vi "JocAcabatSenseSubvis.vi"() -> ()   [LabVIEW 2023]
uses:
  <vilib>/MakerHub/LINX/Public/Peripherals/Analog/Analog Read N Chans.vi
  <vilib>/MakerHub/LINX/Private/Local IO/LinxAnalogRead.vi
  <vilib>/MakerHub/LINX/Public/Utilities/Check Channel.vi
  <vilib>/MakerHub/LINX/Public/Utilities/Open Serial.vi
  <vilib>/MakerHub/LINX/Private/Utilties/Generate Error.vi
  <vilib>/MakerHub/LINX/LMH-LINX.lvlib
panel:
  out "?":string
  out "?":string="Benvingut a la jungla! El teu objectiu és sobreviure! Per aconseguir-ho, has de caçar les preses (punts verds) i fugir dels depredadors (punts vermells). Alerta, a mida que vagis avançant en el joc, aniràn apreixent més preses i depredadors. Per sort, si t'estàs a punt de quedar sense vides, apareixerà un quadrat groc, si l'atrapes, et proporcionarà una vida extra. També has de tenir en compte que tens 40 s per atrapar les preses, si tardes més, et moriràs de gana... Abans que passi però, apareixerà un diamant groc. Atrapa'l i tindràs una mica més de temps per caçar. Bona sort! "
  out "Nivell:":i32
  in  "base path":path
  in  "Serial Port":refnum<visa-resource-name>="N/A"
  out "Tablero":cluster{dbl[], dbl[]}[](graph)
  out "Vides":i32
  out "Preses capturades":i32
  out "Temps sense menjar (s)":u32
  in  "?":bool
  out "ms totals":u32
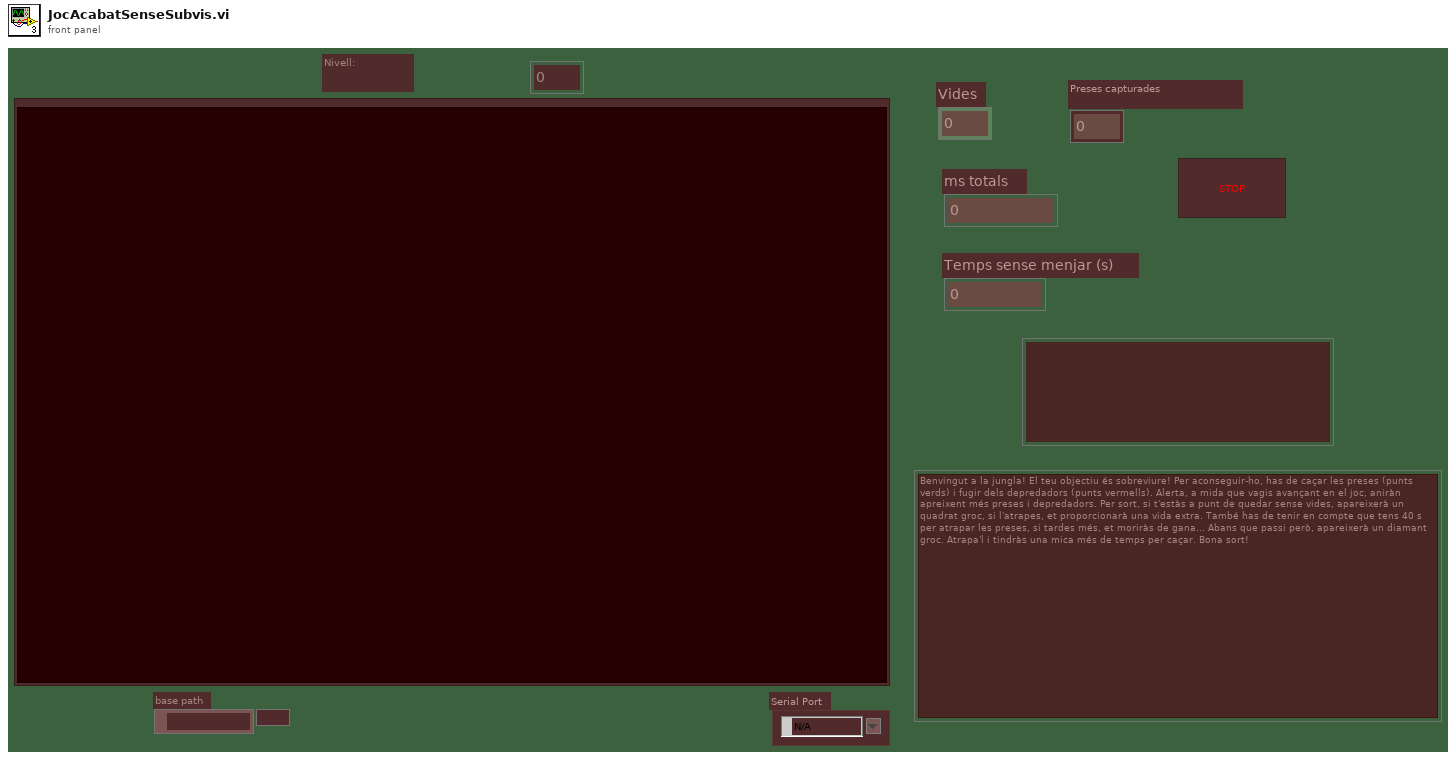
[diagram p1: front panel]
types:
  T1 = enum16{"open", "replace", "create", "open or create", "replace or create", "replace or create with confirmation"}
  T2 = typedef "LMH-LINX.lvlib/LINX Ref.ctl" = cluster{"IO":T3, "Interface":T4, "LINX Device Config":T5}
  T3 = typedef "LMH-LINX.lvlib/Platform.ctl" = enum16{"Remote", "Local"}
  T4 = typedef "LMH-LINX.lvlib/Interface.ctl" = enum16{"Serial", "TCP"}
  T5 = typedef "LMH-LINX.lvlib/Device.lvlib/LINX Device Config.ctl" = cluster{"Interface":T4, "COM Port":refnum<visa-resource-name>, "TCP Configuration":T6, "Device Family":u8, "Device ID":u8, "Device Name":string, "TCP Ref":refnum<k5>, "Channels":T7}
  T6 = typedef "LMH-LINX.lvlib/Device.lvlib/TCP Config.ctl" = cluster{"IP Address":string, "Port":u16}
  T7 = typedef "LMH-LINX.lvlib/Channels.ctl" = cluster{"DI":u8[], "DO":u8[], "AI":u8[], "AO":u8[], "PWM":u8[], "QE":u8[], "UART":u8[], "I2C 2":u8[], "SPI":u8[], "CAN":u8[], "Servo":u8[], "AI Ref (V)":dbl, "AI Resolution (Bits)":u8, "AO Ref (V)":dbl, "AO Resolution (Bits)":u8}
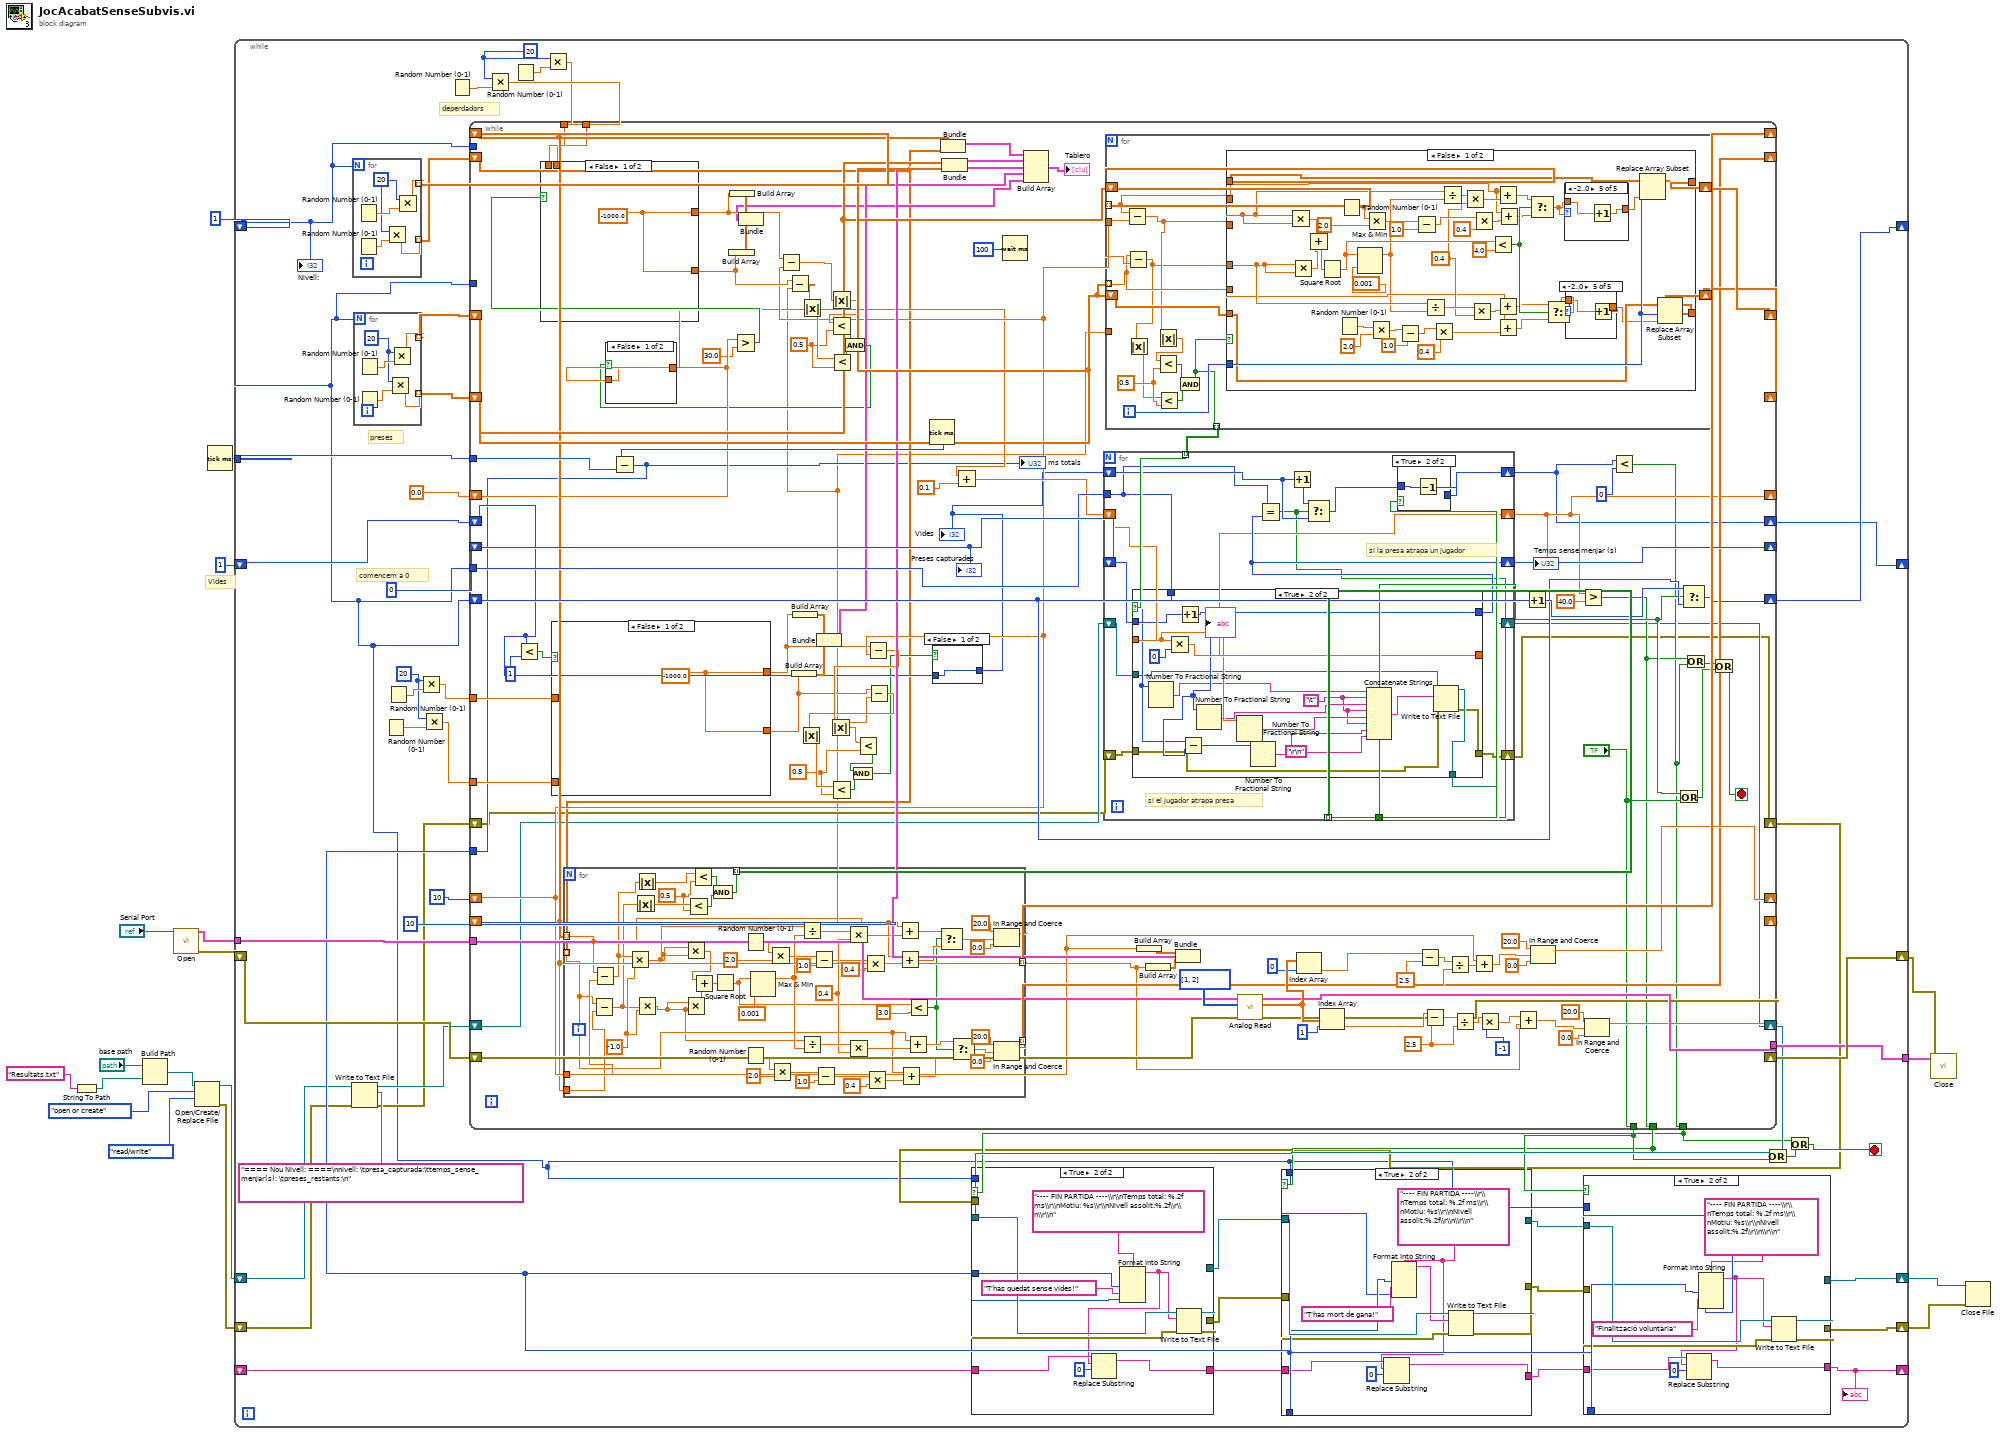
[diagram p0: block diagram]
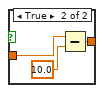
[diagram p5: hidden frame]
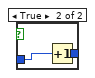
[diagram p6: hidden frame]
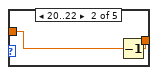
[diagram p8: hidden frame]
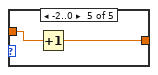
[diagram p11: hidden frame]
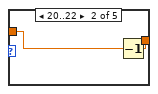
[diagram p12: hidden frame]
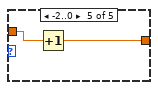
[diagram p15: hidden frame]
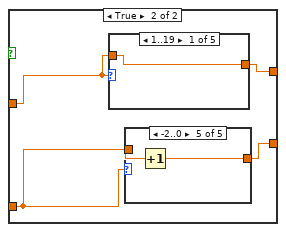
[diagram p16: hidden frame]
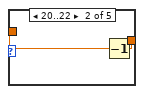
[diagram p18: hidden frame]
diagram:
  # "Vides"
  n1 = String To Path(string="Resultats.txt") -> (path=w3:path)
  n2 = Build Path(base path="base path", name or relative path=w3) -> (appended path=w6:path)
  n3 = call-poly <vilib>:"Open.vi"("Serial Port"="Serial Port") -> ("Error Out"=w12:errorcluster, "LINX Resource"=w13:T2)  [unwired: 8 in, 1 out]
  n4 = Open/Create/Replace File(file path (use dialog)=w6, operation (0:open)=T1."open or create", access (0:read/write)=enum16{"read/write", "read-only", "write-only"}."read/write") -> (refnum out=w9:refnum<file>, error out=w7:errorcluster)  [unwired: 3 in, 1 out]
  n5 = Tick Count (ms)() -> (millisecond timer value=w17:u32)
  n6 = while {
    shift-right: [w63] -> _
    shift-left: 1 -> [w23]
    tunnel: w17 -> [w54]
    shift-right: [w60] -> _
    shift-left: 1 -> [w61]
    tunnel: [w58] -> w14
    tunnel: w13 -> [w57]
    shift-right: [w59] -> w15
    shift-left: w12 -> [w55]
    shift-right: [w25] -> w2
    shift-left: w7 -> [w30]
    shift-right: [w24] -> w1
    shift-left: w9 -> [w33]
    shift-right: [w19] -> _
    shift-left: _ -> [w22]
    stop <- w40 stop-if-true
    w44 = 20
    w47 = 20
    # "comencem a 0"
    # "deperdadors"
    # "preses"
    n7 = Write to Text File(file (use dialog)=w33, text="==== Nou Nivell: ====\nnivell: \tpresa_capturada:\ttemps_sense_menjar(s): \tpreses_restants:\n", error in=w30) -> (refnum out=w34:refnum<file>, error out=w29:errorcluster)  [unwired: 1 in, 1 out]
    n8 = for {
      N: w23 -> [_]
      tunnel: [w450] -> w68 mode=indexing
      tunnel: [w449] -> w67 mode=indexing
      w451 = 20
      n9 = Random Number (0-1)() -> (number: 0 to 1=w453:dbl)
      n10 = Random Number (0-1)() -> (number: 0 to 1=w452:dbl)
      n11 = Multiply(x=w451, y=w452) -> (x*y=w449:dbl)
      n12 = Multiply(x=w451, y=w453) -> (x*y=w450:dbl)
    }
    n13 = for {
      N: w23 -> [_]
      tunnel: [w445] -> w66 mode=indexing
      tunnel: [w444] -> w65 mode=indexing
      w446 = 20
      n14 = Random Number (0-1)() -> (number: 0 to 1=w448:dbl)
      n15 = Random Number (0-1)() -> (number: 0 to 1=w447:dbl)
      n16 = Multiply(x=w446, y=w447) -> (x*y=w444:dbl)
      n17 = Multiply(x=w446, y=w448) -> (x*y=w445:dbl)
    }
    n18 = Random Number (0-1)() -> (number: 0 to 1=w46:dbl)
    n19 = Random Number (0-1)() -> (number: 0 to 1=w45:dbl)
    n20 = Multiply(x=w44, y=w45) -> (x*y=w42:dbl)
    n21 = Multiply(x=w44, y=w46) -> (x*y=w43:dbl)
    n22 = Random Number (0-1)() -> (number: 0 to 1=w51:dbl)
    n23 = Multiply(x=w47, y=w51) -> (x*y=w49:dbl)
    n24 = Random Number (0-1)() -> (number: 0 to 1=w50:dbl)
    n25 = Multiply(x=w47, y=w50) -> (x*y=w48:dbl)
    n26 = while {
      tunnel: w23 -> [_]
      shift-right: [w202] -> _
      shift-left: w68 -> [w163]
      shift-right: [w183] -> _
      shift-left: w67 -> [w125]
      shift-right: [w192] -> _
      shift-left: w66 -> [w186]
      shift-right: [w185] -> _
      shift-left: w65 -> [w193]
      shift-right: [w198] -> _
      shift-left: 10 -> [w140]
      shift-right: [w194] -> _
      shift-left: 10 -> [w114]
      shift-right: [w203] -> w59
      shift-left: w55 -> [w205]
      tunnel: [w204] -> w58
      tunnel: w23 -> [_]
      shift-right: [w170] -> w60
      shift-left: w61 -> [w138]
      shift-right: [w188] -> _
      shift-left: 0 -> [w190]
      tunnel: w23 -> [w184]
      tunnel: [w171] -> w37
      shift-right: [w180] -> w63
      shift-left: w23 -> [w181]
      tunnel: w57 -> [w179]
      tunnel: ["?"] -> w38
      tunnel: w54 -> [w176]
      shift-right: [w173] -> _
      shift-left: 0.0 -> [w135]
      tunnel: [w165] -> w36
      tunnel: w49 -> [w124]
      tunnel: w48 -> [w123]
      tunnel: w43 -> [w122]
      tunnel: w42 -> [w121]
      shift-right: [w118] -> w39
      shift-left: w34 -> [w119]
      tunnel: [w117] -> w35
      shift-right: [w115] -> w28
      shift-left: w29 -> [w116]
      stop <- w166 stop-if-true
      w133 = 0.5
      w132 = 0.5
      w213 = 2.5
      w214 = 2.5
      n27 = Less?(x=w138, y=1) -> (x < y?=w161:bool)
      n28 = case shown="False" w161 {
        tunnel: [w249 w253] -> w129
        tunnel: [w249 w252] -> w139
        tunnel: w122 -> [_ w251]
        tunnel: w121 -> [_ w250]
        frame False {
          w249 = -1000.0
        }
        frame True {
          n29 = case shown="1..19" w250 {
            tunnel: [w261 w263 w264 w265 w267] -> w253
            tunnel: w250 -> [w261 w262 w264 w265 w266]
            frame 1..19 {
            }
            frame 20..22 {
              n30 = Decrement(x=w262) -> (x-1=w263:dbl)
            }
            frame 23.. {
            }
            frame ..-3 {
            }
            frame -2..0 {
              n31 = Increment(x=w266) -> (x+1=w267:dbl)
            }
          }
          n32 = case shown="-2..0" w251 {
            tunnel: [w254 w256 w257 w258 w260] -> w252
            tunnel: w251 -> [w254 w255 w257 w258 w259]
            frame 1..19 {
            }
            frame 20..22 {
              n33 = Decrement(x=w255) -> (x-1=w256:dbl)
            }
            frame 23.. {
            }
            frame ..-3 {
            }
            frame -2..0 {
              n34 = Increment(x=w259) -> (x+1=w260:dbl)
            }
          }
        }
      }
      n35 = for {
        tunnel: w140 -> [w325]
        tunnel: w114 -> [w324]
        tunnel: w125 -> [w319] mode=indexing
        tunnel: w163 -> [w320] mode=indexing
        tunnel: [w323] -> w202 mode=indexing
        tunnel: [w322] -> w183 mode=indexing
        tunnel: [w309] -> w189 mode=indexing
        w312 = 0.5
        w321 = -1.0
        w355 = 0.4
        n36 = Subtract(x=w319, y=w324) -> (x-y=w315:dbl)
        n37 = Subtract(x=w320, y=w325) -> (x-y=w316:dbl)
        n38 = Multiply(x=w316, y=w321) -> (x*y=w318:dbl)
        n39 = Absolute Value(x=w315) -> (abs(x)=w313:dbl)
        n40 = Absolute Value(x=w316) -> (abs(x)=w314:dbl)
        n41 = Multiply(x=w315, y=w321) -> (x*y=w317:dbl)
        n42 = Multiply(x=w318, y=w318) -> (x*y=w362:dbl)
        n43 = Multiply(x=w317, y=w317) -> (x*y=w361:dbl)
        n44 = Less?(x=w313, y=w312) -> (x < y?=w310:bool)
        n45 = Less?(x=w314, y=w312) -> (x < y?=w311:bool)
        n46 = Add(x=w362, y=w361) -> (x+y=w360:dbl)
        n47 = And(x=w311, y=w310) -> (x .and. y?=w309:bool)
        n48 = Square Root(x=w360) -> (sqrt(x)=w326:dbl)
        n49 = Random Number (0-1)() -> (number: 0 to 1=w344:dbl)
        n50 = Random Number (0-1)() -> (number: 0 to 1=w351:dbl)
        n51 = Max & Min(x=w326, y=0.001) -> (max(x,y)=w357:dbl)  [unwired: 1 out]
        n52 = Multiply(x=w344, y=2.0) -> (x*y=w342:dbl)
        n53 = Multiply(x=w351, y=2.0) -> (x*y=w349:dbl)
        n54 = Divide(x=w318, y=w357) -> (x/y=w354:dbl)
        n55 = Divide(x=w317, y=w357) -> (x/y=w356:dbl)
        n56 = Subtract(x=w342, y=1.0) -> (x-y=w340:dbl)
        n57 = Subtract(x=w349, y=1.0) -> (x-y=w347:dbl)
        n58 = Multiply(x=w354, y=w355) -> (x*y=w353:dbl)
        n59 = Multiply(x=w356, y=w355) -> (x*y=w352:dbl)
        n60 = Multiply(x=w340, y=0.4) -> (x*y=w338:dbl)
        n61 = Multiply(x=w347, y=0.4) -> (x*y=w345:dbl)
        n62 = Add(x=w320, y=w353) -> (x+y=w334:dbl)
        n63 = Add(x=w320, y=w338) -> (x+y=w335:dbl)
        n64 = Add(x=w319, y=w345) -> (x+y=w337:dbl)
        n65 = Add(x=w319, y=w352) -> (x+y=w336:dbl)
        n66 = Less?(x=w326, y=3.0) -> (x < y?=w333:bool)
        n67 = Select(t=w334, s=w333, f=w335) -> (s? t:f=w331:dbl)
        n68 = Select(t=w336, s=w333, f=w337) -> (s? t:f=w332:dbl)
        n69 = In Range and Coerce(upper limit=20.0, x=w331, lower limit=0.0) -> (coerced(x)=w323:dbl)  [unwired: 1 out]
        n70 = In Range and Coerce(upper limit=20.0, x=w332, lower limit=0.0) -> (coerced(x)=w322:dbl)  [unwired: 1 out]
      }
      n71 = Greater?(x=w135, y=30.0) -> (0:w157:bool)
      n72 = case shown="False" w157 {
        tunnel: [w230 w234] -> w149
        tunnel: [w230 w233] -> w148
        tunnel: w124 -> [_ w232]
        tunnel: w123 -> [_ w231]
        frame False {
          w230 = -1000.0
        }
        frame True {
          n73 = case shown="1..19" w231 {
            tunnel: [w242 w244 w245 w246 w248] -> w234
            tunnel: w231 -> [w242 w243 w245 w246 w247]
            frame 1..19 {
            }
            frame 20..22 {
              n74 = Decrement(x=w243) -> (x-1=w244:dbl)
            }
            frame 23.. {
            }
            frame ..-3 {
            }
            frame -2..0 {
              n75 = Increment(x=w247) -> (x+1=w248:dbl)
            }
          }
          n76 = case shown="1..19" w232 {
            tunnel: [w235 w237 w238 w239 w241] -> w233
            tunnel: w232 -> [w235 w236 w238 w239 w240]
            frame 1..19 {
            }
            frame 20..22 {
              n77 = Decrement(x=w236) -> (x-1=w237:dbl)
            }
            frame 23.. {
            }
            frame ..-3 {
            }
            frame -2..0 {
              n78 = Increment(x=w240) -> (x+1=w241:dbl)
            }
          }
        }
      }
      n79 = Build Array(w148) -> (w155:dbl[])
      n80 = Build Array(w149) -> (w156:dbl[])
      n81 = Bundle(w156, w155) -> (w131:cluster{dbl[], dbl[]})  [unwired: 1 in]
      n82 = Subtract(x=w149, y=w140) -> (x-y=w147:dbl)
      n83 = Subtract(x=w148, y=w114) -> (x-y=w150:dbl)
      n84 = Build Array(w139) -> (w159:dbl[])
      n85 = Build Array(w129) -> (w160:dbl[])
      n86 = Absolute Value(x=w150) -> (abs(x)=w152:dbl)
      n87 = Bundle(w160, w159) -> (w158:cluster{dbl[], dbl[]})  [unwired: 1 in]
      n88 = Absolute Value(x=w147) -> (abs(x)=w151:dbl)
      n89 = Less?(x=w151, y=w132) -> (x < y?=w154:bool)
      n90 = Less?(x=w152, y=w132) -> (x < y?=w153:bool)
      n91 = And(x=w154, y=w153) -> (x .and. y?=w128:bool)
      n92 = case shown="False" w128 {
        tunnel: w135 -> [w223 w226]
        tunnel: [w223 w224] -> w134
        frame False {
        }
        frame True {
          n93 = Subtract(x=w226, y=10.0) -> (x-y=w224:dbl)
        }
      }
      n94 = Subtract(x=w129, y=w140) -> (x-y=w144:dbl)
      n95 = Absolute Value(x=w144) -> (abs(x)=w143:dbl)
      n96 = Less?(x=w143, y=w133) -> (x < y?=w146:bool)
      n97 = Subtract(x=w139, y=w114) -> (x-y=w142:dbl)
      n98 = Absolute Value(x=w142) -> (abs(x)=w141:dbl)
      n99 = Less?(x=w141, y=w133) -> (x < y?=w145:bool)
      n100 = And(x=w146, y=w145) -> (x .and. y?=w137:bool)
      n101 = Tick Count (ms)() -> (millisecond timer value=w177:u32)
      n102 = Subtract(x=w177, y=w176) -> (x-y=w117:u32)
      "ms totals" <- w117
      n103 = case shown="False" w137 {
        tunnel: w138 -> [w227 w229]
        tunnel: [w227 w228] -> w136
        frame False {
        }
        frame True {
          n104 = Increment(x=w229) -> (x+1=w228:i32)
        }
      }
      "Vides" <- w136
      n105 = Bundle(w163, w125) -> (w191:cluster{dbl[], dbl[]})  [unwired: 1 in]
      n106 = Bundle(w186, w193) -> (w126:cluster{dbl[], dbl[]})  [unwired: 1 in]
      n107 = Add(x=w134, y=0.1) -> (x+y=w174:dbl)
      n108 = Wait (ms)(milliseconds to wait=u32 100) -> ()  [unwired: 1 out]
      n109 = for {
        tunnel: w140 -> [w379]
        tunnel: w114 -> [w374]
        tunnel: w186 -> [w373] mode=indexing
        tunnel: w193 -> [w369] mode=indexing
        shift-right: [w368] -> w192
        shift-left: w186 -> [w372]
        shift-right: [w370] -> w185
        shift-left: w193 -> [w371]
        tunnel: [w363] -> w120 mode=indexing
        i -> [w378]
        w377 = 0.5
        n110 = Subtract(x=w373, y=w379) -> (x-y=w366:dbl)
        n111 = Subtract(x=w369, y=w374) -> (x-y=w364:dbl)
        n112 = Absolute Value(x=w364) -> (abs(x)=w367:dbl)
        n113 = Absolute Value(x=w366) -> (abs(x)=w365:dbl)
        n114 = Less?(x=w365, y=w377) -> (x < y?=w376:bool)
        n115 = Less?(x=w367, y=w377) -> (x < y?=w375:bool)
        n116 = And(x=w376, y=w375) -> (x .and. y?=w363:bool)
        n117 = case shown="False" w363 {
          tunnel: w378 -> [w386 w438]
          tunnel: w373 -> [w391 _]
          tunnel: w369 -> [w393 _]
          tunnel: w366 -> [w392 _]
          tunnel: w364 -> [w394 _]
          tunnel: w372 -> [w390 w442]
          tunnel: w371 -> [w382 w443]
          tunnel: [w389 w441] -> w368
          tunnel: [w388 w440] -> w370
          frame False {
            w397 = 0.4
            n118 = Multiply(x=w392, y=w392) -> (x*y=w404:dbl)
            n119 = Multiply(x=w394, y=w394) -> (x*y=w405:dbl)
            n120 = Add(x=w404, y=w405) -> (x+y=w406:dbl)
            n121 = Square Root(x=w406) -> (sqrt(x)=w407:dbl)
            n122 = Random Number (0-1)() -> (number: 0 to 1=w412:dbl)
            n123 = Random Number (0-1)() -> (number: 0 to 1=w416:dbl)
            n124 = Max & Min(x=w407, y=0.001) -> (max(x,y)=w384:dbl)  [unwired: 1 out]
            n125 = Multiply(x=w416, y=2.0) -> (x*y=w417:dbl)
            n126 = Multiply(x=w412, y=2.0) -> (x*y=w413:dbl)
            n127 = Subtract(x=w413, y=1.0) -> (x-y=w414:dbl)
            n128 = Subtract(x=w417, y=1.0) -> (x-y=w418:dbl)
            n129 = Divide(x=w394, y=w384) -> (x/y=w408:dbl)
            n130 = Multiply(x=w414, y=0.4) -> (x*y=w415:dbl)
            n131 = Divide(x=w392, y=w384) -> (x/y=w409:dbl)
            n132 = Multiply(x=w409, y=w397) -> (x*y=w410:dbl)
            n133 = Multiply(x=w408, y=w397) -> (x*y=w411:dbl)
            n134 = Multiply(x=w418, y=0.4) -> (x*y=w419:dbl)
            n135 = Less?(x=w407, y=4.0) -> (x < y?=w423:bool)
            n136 = Add(x=w391, y=w410) -> (x+y=w387:dbl)
            n137 = Add(x=w393, y=w411) -> (x+y=w421:dbl)
            n138 = Add(x=w393, y=w415) -> (x+y=w420:dbl)
            n139 = Add(x=w391, y=w419) -> (x+y=w422:dbl)
            n140 = Select(t=w387, s=w423, f=w422) -> (s? t:f=w383:dbl)
            n141 = Select(t=w421, s=w423, f=w420) -> (s? t:f=w381:dbl)
            n142 = case shown="-2..0" w383 {
              tunnel: [w431 w432 w434 w435 w437] -> w385
              tunnel: w383 -> [w431 w433 w434 w435 w436]
              frame 1..19 {
              }
              frame 20..22 {
                n143 = Decrement(x=w433) -> (x-1=w432:dbl)
              }
              frame 23.. {
              }
              frame ..-3 {
              }
              frame -2..0 {
                n144 = Increment(x=w436) -> (x+1=w437:dbl)
              }
            }
            n145 = case shown="-2..0" w381 {
              tunnel: [w424 w425 w427 w428 w430] -> w380
              tunnel: w381 -> [w424 w426 w427 w428 w429]
              frame 1..19 {
              }
              frame 20..22 {
                n146 = Decrement(x=w426) -> (x-1=w425:dbl)
              }
              frame 23.. {
              }
              frame ..-3 {
              }
              frame -2..0 {
                n147 = Increment(x=w429) -> (x+1=w430:dbl)
              }
            }
            n148 = Replace Array Subset(array=w390, new element=w385, index=w386) -> (w389:dbl[])
            n149 = Replace Array Subset(array=w382, new element=w380, index=w386) -> (w388:dbl[])
          }
          frame True {
            w439 = -1000
            n150 = Replace Array Subset(array=w443, new element=w439, index=w438) -> (w440:dbl[])
            n151 = Replace Array Subset(array=w442, new element=w439, index=w438) -> (w441:dbl[])
          }
        }
      }
      n152 = for {
        tunnel: w120 -> [w281] mode=indexing
        shift-right: [w276] -> w188
        shift-left: w190 -> [w280]
        tunnel: w184 -> [w271]
        shift-right: [w277] -> w170
        shift-left: w136 -> [w279]
        tunnel: w189 -> [w278] mode=indexing
        shift-right: [w275] -> w173
        shift-left: w174 -> [w274]
        tunnel: [w273] -> w172
        shift-right: [w268] -> w115
        shift-left: w116 -> [w269]
        shift-right: [w270] -> w118
        shift-left: w119 -> [w272]
        # "si la presa atrapa un jugador"
        # "si el jugador atrapa presa"
        n153 = case shown="True" w281 {
          tunnel: [w290 w304] -> w276
          tunnel: w280 -> [w290 w308]
          tunnel: w274 -> [w289 w305]
          tunnel: [w289 w307] -> w275
          tunnel: w272 -> [w288 w296]
          tunnel: w271 -> [_ w298]
          tunnel: [w288 w302] -> w270
          tunnel: w269 -> [w287 w301]
          tunnel: [w287 w300] -> w268
          frame False {
          }
          frame True {
            w293 = "\t"
            n154 = Number To Fractional String(number=w298) -> (F-format string=w297:string)  [unwired: 3 in]
            n155 = Multiply(x=w305, y=0) -> (x*y=w307:dbl)
            n156 = Increment(x=w308) -> (x+1=w304:i32)
            n157 = Subtract(x=w298, y=w304) -> (x-y=w303:i32)
            n158 = Number To Fractional String(number=w304) -> (F-format string=w295:string)  [unwired: 3 in]
            n159 = Number To Fractional String(number=w305) -> (F-format string=w294:string)  [unwired: 3 in]
            n160 = Number To Fractional String(number=w303) -> (F-format string=w292:string)  [unwired: 3 in]
            n161 = Concatenate Strings(w297, w293, w295, w293, w294, w293, w292, "\r\n") -> (w299:string)
            n162 = Write to Text File(file (use dialog)=w296, text=w299, error in=w301) -> (refnum out=w302:refnum<file>, error out=w300:errorcluster)  [unwired: 1 in, 1 out]
          }
        }
        n163 = Equal?(x=w271, y=w276) -> (x = y?=w273:bool)
        n164 = Increment(x=w279) -> (x+1=w283:i32)
        n165 = Select(t=w283, s=w273, f=w279) -> (s? t:f=w282:i32)
        n166 = case shown="True" w278 {
          tunnel: w282 -> [w284 w286]
          tunnel: [w284 w285] -> w277
          frame False {
          }
          frame True {
            n167 = Decrement(x=w286) -> (x-1=w285:i32)
          }
        }
      }
      "Temps sense menjar (s)" <- w173
      n168 = Build Array(w140) -> (w220:dbl[])
      n169 = Build Array(w114) -> (w210:dbl[])
      n170 = Bundle(w220, w210) -> (w162:cluster{dbl[], dbl[]})  [unwired: 1 in]
      n171 = Build Array(w191, w126, w162, w158, w131) -> (→"Tablero":cluster{dbl[], dbl[]}[])
      n172 = call-poly <vilib>:"Analog Read.vi"("Error In"=w205, "AI Channel(s)"=u8[] [1, 2], "LINX Resource"=w179) -> ("Error Out"=w203:errorcluster, "Voltages"=w218:dbl[], "LINX Resource"=w204:T2)  [unwired: 5 in, 1 out]
      n173 = Index Array(array=w218, index=0) -> (element=w216:dbl)
      n174 = Index Array(array=w218, index=1) -> (element=w215:dbl)
      n175 = Subtract(x=w216, y=w214) -> (x-y=w221:dbl)
      n176 = Subtract(x=w215, y=w213) -> (x-y=w208:dbl)
      n177 = Divide(x=w221, y=w214) -> (x/y=w212:dbl)
      n178 = Divide(x=w208, y=w213) -> (x/y=w207:dbl)
      n179 = Add(x=w140, y=w212) -> (x+y=w199:dbl)
      n180 = Multiply(x=w207, y=-1) -> (x*y=w206:dbl)
      n181 = Add(x=w206, y=w114) -> (x+y=w195:dbl)
      n182 = Increment(x=w181) -> (x+1=w182:i32)
      n183 = In Range and Coerce(upper limit=20.0, x=w199, lower limit=0.0) -> (coerced(x)=w198:dbl)  [unwired: 1 out]
      n184 = Greater?(x=w173, y=40.0) -> (0:w171:bool)
      n185 = In Range and Coerce(upper limit=20.0, x=w195, lower limit=0.0) -> (coerced(x)=w194:dbl)  [unwired: 1 out]
      n186 = Less?(x=w170, y=0) -> (x < y?=w165:bool)
      n187 = Or(x=w172, y="?") -> (x .or. y?=w167:bool)
      n188 = Select(t=w182, s=w172, f=w181) -> (s? t:f=w180:i32)
      n189 = Or(x=w171, y=w165) -> (x .or. y?=w168:bool)
      n190 = Or(x=w168, y=w167) -> (x .or. y?=w166:bool)
      "Preses capturades" <- w190
    }
    n191 = case shown="True" w36 {
      tunnel: w39 -> [w101 w112]
      tunnel: w35 -> [_ w110]
      tunnel: [w101 w109] -> w32
      tunnel: w28 -> [w100 w108]
      tunnel: [w100 w107] -> w27
      tunnel: w23 -> [_ w106]
      tunnel: w22 -> [w99 w105]
      tunnel: [w99 w104] -> w21
      frame False {
      }
      frame True {
        n192 = Format Into String(format string="---- FIN PARTIDA ----\\r\\nTemps total: %.2f ms\\r\\nMotiu: %s\\r\\nNivell assolit:%.2f\\r\\n\\r\\n", w110, "T'has quedat sense vides!", w106) -> (resulting string=w103:string)  [unwired: 2 in, 1 out]
        n193 = Replace Substring(3:0 ("offset (0)"), 4:w103, 5:w105) -> (1:w104:string)  [unwired: 1 in, 1 out]
        n194 = Write to Text File(file (use dialog)=w112, text=w103, error in=w108) -> (refnum out=w109:refnum<file>, error out=w107:errorcluster)  [unwired: 1 in, 1 out]
      }
    }
    n195 = case shown="True" w37 {
      tunnel: w32 -> [w86 w98]
      tunnel: w35 -> [_ w95]
      tunnel: [w86 w94] -> w31
      tunnel: w27 -> [w85 w93]
      tunnel: [w85 w92] -> w26
      tunnel: w23 -> [_ w91]
      tunnel: w21 -> [w84 w90]
      tunnel: [w84 w89] -> w20
      frame False {
      }
      frame True {
        w88 = "---- FIN PARTIDA ----\\r\\nTemps total: %.2f ms\\r\\nMotiu: %s\\r\\nNivell assolit:%.2f\\r\\n\\r\\n"
        n196 = Replace Substring(3:0 ("offset (0)"), 4:w88, 5:w90) -> (1:w89:string)  [unwired: 1 in, 1 out]
        n197 = Format Into String(format string=w88, w95, "T'has mort de gana!", w91) -> (resulting string=w97:string)  [unwired: 2 in, 1 out]
        n198 = Write to Text File(file (use dialog)=w98, text=w97, error in=w93) -> (refnum out=w94:refnum<file>, error out=w92:errorcluster)  [unwired: 1 in, 1 out]
      }
    }
    n199 = case shown="True" w38 {
      tunnel: w31 -> [w71 w83]
      tunnel: w35 -> [_ w81]
      tunnel: [w71 w80] -> w24
      tunnel: w26 -> [w70 w79]
      tunnel: [w70 w78] -> w25
      tunnel: w23 -> [_ w77]
      tunnel: w20 -> [w69 w75]
      tunnel: [w69 w74] -> w19
      frame False {
      }
      frame True {
        n200 = Format Into String(format string="---- FIN PARTIDA ----\\r\\nTemps total: %.2f ms\\r\\nMotiu: %s\\r\\nNivell assolit:%.2f\\r\\n\\r\\n", w81, "Finalització voluntària", w77) -> (resulting string=w73:string)  [unwired: 2 in, 1 out]
        n201 = Replace Substring(3:0 ("offset (0)"), 4:w73, 5:w75) -> (1:w74:string)  [unwired: 1 in, 1 out]
        n202 = Write to Text File(file (use dialog)=w83, text=w73, error in=w79) -> (refnum out=w80:refnum<file>, error out=w78:errorcluster)  [unwired: 1 in, 1 out]
      }
    }
    "?" <- w19
    n203 = Or(x=w37, y=w38) -> (x .or. y?=w52:bool)
    n204 = Or(x=w36, y=w52) -> (x .or. y?=w40:bool)
    "Nivell:" <- w23
  }
  n205 = call <vilib>:"Close.vi"("Error In"=w15, "LINX Resource"=w14) -> ()  [unwired: 9 in, 1 out]
  n206 = Close File(refnum=w1, error in=w2) -> ()  [unwired: 2 out]
